vi "FuncVI-Mode.vi"(5 "InstanceRef":T2, 9 "arg list":T1[](array[typedef]) {"num" format="%.2f"}) -> (0 "error out":bool, 3 "result":T1 {"num" format="%.2f"})   [LabVIEW 2021]
doc: "::: CalcExpress Toolkit :::\nCopyright (c) 2000-2026 Konstantin Shifershteyn. All rights reserved."
uses:
  cetypes.llb/CalcExpress Function Argument Info.ctl
  cetypes.llb/CalcExpress Instance RefNum.ctl
  <vilib>/Analysis/baseanly.llb/Unimode.vi
  <vilib>/Analysis/NI_AALBase.lvlib
panel:
  in  "max arg num":i32=2
  in  "min arg num":i32=1
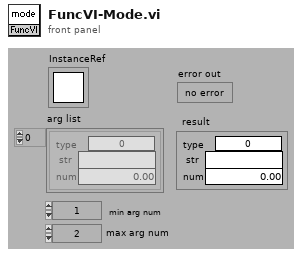
[diagram p1: front panel]
types:
  T1 = typedef "CalcExpress Function Argument Info.ctl" = cluster{"type":u32, "str":string, "num":dbl}
  T2 = typedef "CalcExpress Instance RefNum.ctl" = refnum<k1>
  T3 = enum32{"String", "DBL Number", "identifier", "1D Array of DBL", "2D Array of DBL", "CDB Number", "1D Array of CDB", "2D Array of CDB", "1D Array of String", "2D Array of String", "Unknown data type"}
  T4 = cluster{"use this constant to specify a predefined type":enum32{"String", "DBL Number", "identifier", "1D Array of DBL", "2D Array of DBL", "CDB Number", "1D Array of CDB", "2D Array of CDB", "1D Array of String", "2D Array of String", "Unknown data type"}, string, "mode":dbl}
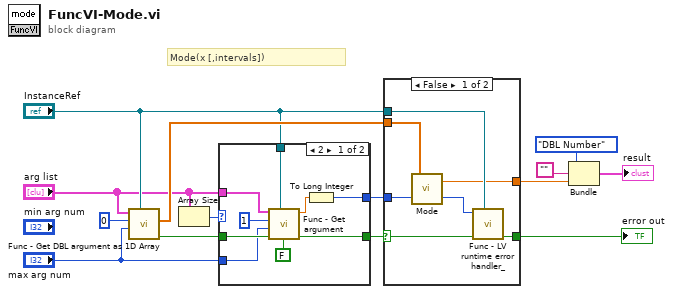
[diagram p0: block diagram]
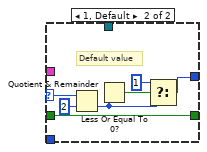
[diagram p2: hidden frame]
diagram:
  # "Mode(x [,intervals])"
  n1 = call "Func - Get DBL argument as 1D Array.vi"("InstanceRef"="InstanceRef", "max arg num"="max arg num", "arg idx"=0, "arg list"="arg list") -> ("error out"=w7:bool, "1D data"=w14:dbl[])  [unwired: 4 in, 2 out]
  n2 = Array Size(array="arg list") -> (size(s)=w3:i32)
  n3 = case shown="2" w3 {
    selector: w3 -> [_ w29]
    tunnel: w7 -> [w23 w30]
    tunnel: [w22 w30] -> w6
    tunnel: "InstanceRef" -> [w21 _]
    tunnel: "max arg num" -> [w19 _]
    tunnel: "arg list" -> [w17 _]
    tunnel: [w15 w24] -> w4
    frame 2 {
      n4 = call "Func - Get argument.vi"("ena NonNum? (F)"=FALSE, "InstanceRef"=w21, "error in"=w23, "max arg num"=w19, "arg idx"=1, "arg list"=w17) -> ("error out"=w22:bool, "num"=w16:dbl)  [unwired: 2 out]
      n5 = To Long Integer(number=w16) -> (32bit integer=w15:i32)
    }
    frame 1, Default {
      # "Default value"
      n6 = Quotient & Remainder(x=w29, y=2) -> (floor(x/y)=w27:i32)  [unwired: 1 out]
      n7 = Less Or Equal To 0?(x=w27) -> (x <= 0?=w26:bool)
      n8 = Select(t=1, s=w26, f=w27) -> (s? t:f=w24:i32)
    }
  }
  n9 = case shown="False" w6 {
    selector: w6 -> [w37 w38]
    tunnel: w14 -> [w32 _]
    tunnel: [w33 _] -> w8
    tunnel: [w36 w38] -> w12
    tunnel: "InstanceRef" -> [w35 _]
    tunnel: w4 -> [w31 _]
    frame False {
      n10 = call-poly <vilib>:"Mode.vi"("intervals"=w31, "X"=w32) -> ("error"=w34:i32, "mode"=w33:dbl)
      n11 = call "Func - LV runtime error handler_.vi"("InstanceRef"=w35, "error in"=w37, "LabVIEW error code"=w34) -> ("error out"=w36:bool)  [unwired: 8 in]
    }
    frame True {
    }
  }
  "error out" <- w12
  n12 = Bundle("use this constant to specify a predefined type"=T3."DBL Number", "", "mode"=w8) -> (→"result":T4)  [unwired: 1 in]
